vi "K_S30 Global.vi"() -> ()   [LabVIEW 2022 SP3]
panel:
  in  "RS-converter:\necho":bool=TRUE
  in  "VISA resource":refnum<visa-resource-name>="COM2"
  # "Global Variable for KELLER S30 driver Labview"
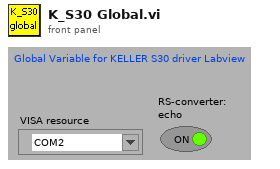
[diagram p1: front panel]
diagram:
